vi "Control - Industrial Control.vi"() -> ()   [LabVIEW 2019, in "Control Workspace Object.lvlib"]
doc: "Sample numeric display item."
uses:
  Control Workspace Object.lvlib
  <vilib>/NI VeriStand/Display Template Support/DisplayTemplateSupport.llb/enum_Display Template Handler Minimal To Widget Msg.ctl
  <vilib>/NI VeriStand/Display Template Support/DisplayTemplateSupport.llb/enum_Display Template Handler Minimal To Workspace.ctl
  Addon/Addon Shared/SubVIs/Constants.vi
  Addon/Addon Shared/Control Addon Shared.lvlib
  Workspace Shared/Control Workspace Shared.lvlib
  Types/Workspace Object Cached Settings.ctl
  Types/Workspace Object State Variables.ctl
  <vilib>/NI VeriStand/Execution/Workspace/NI_VS Workspace ExecutionAPI.lvlib
  Workspace Shared/Types/UDP Streaming Command Cluster.ctl
  Workspace Shared/Types/UDP Streaming State.ctl
  <vilib>/NI VeriStand/Execution/Workspace/SystemStateRegEventRef.ctl
  <vilib>/NI VeriStand/Execution/Workspace/WorkspaceAPI.ctl
  <vilib>/NI VeriStand/Execution/Workspace/SystemStateEventRef.ctl
  Workspace Shared/Types/UI.Chart.Refs.ctl
  <vilib>/NI VeriStand/Execution/Workspace/Target State.ctl
  <vilib>/NI VeriStand/Execution/Workspace/Target State Info.ctl
  <vilib>/NI VeriStand/Execution/Workspace/NI VeriStand - Get Multiple Channel Values.vi
  <vilib>/NI VeriStand/Display Template Support/DisplayTemplateSupport.llb/sub_Display Template Handler Custom.vi
  <vilib>/NI VeriStand/Execution/Workspace/NI VeriStand - Set Single Channel Value.vi
  NationalInstruments.VeriStand.ClientAPI
  NationalInstruments.VeriStand.SystemStorage
  <vilib>/NI VeriStand/Display Template Support/DisplayTemplateSupport.llb/cluster_Screen Item Settings.ctl
  <vilib>/NI VeriStand/Display Template Support/DisplayTemplateSupport.llb/cluster_Graph Scale Settings.ctl
  <vilib>/NI VeriStand/Display Template Support/DisplayTemplateSupport.llb/cluster_Graph Plot Settings.ctl
panel:
  in  "Manual Value":bool
  in  "Revert":bool
  in  "Apply":bool
  in  "Manual Output":dbl
  in  "Manual Control":bool
  in  "Setpoint":dbl
  in  "NIVS.System Definition Root":refnum<k24>
  in  "NIVS.Gateway IP Address":string
  in  "Hold":bool
  in  "Autoscale Y":bool=TRUE
  in  "Autoscale X":bool=TRUE
  out "Chart":waveform(dbl)[](graph)
  out "Device":string
  in  "Item.Data":T1
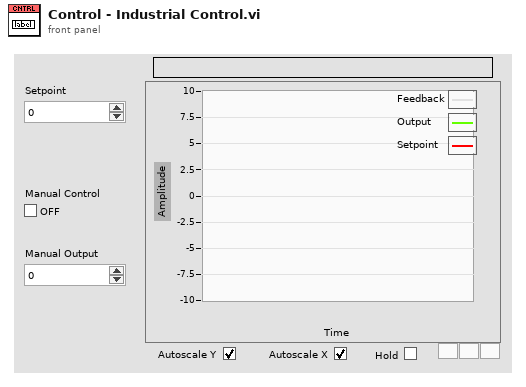
[diagram p1: front panel]
types:
  T1 = typedef "cluster_Screen Item Settings.ctl" = cluster{"Template VI":string, "Position X":i32, "Position Y":i32, "Custom":string, "Show Title Bar":bool, "ID":i32, "Always On Top":bool, "Allow Resize":bool, "Allow Minimize":bool, "Allow Close":bool, "Size to Screen":bool, "Screen.ID":i32, "State":enum16{"Normal", "New"}, "Title":string, "Window Bounds":cluster{"[0]":i16, "[1]":i16, "[2]":i16, "[3]":i16}, "Channel Ref":u64, "Unit":string, "Default Units?":bool, "Flash Limit?":bool, "Color 1":u32, "Color 2":u32, "Color 3":u32, "Color 4":u32, "Bck Color":u32, "Fore Color":u32, "Limit 1":dbl, "Limit 2":dbl, "Limit 3":dbl, "Limit 4":dbl, "Limit Mode 1":i32, "Limit Mode 2":i32, "Limit Mode 3":i32, "Limit Mode 4":i32, "Scale Precision":i32, "Scale Min":dbl, "Scale Max":dbl, "Format":i32, "Precision":i32, "Background Type":i32, "IDs":i32[], "Units":string[], "Labels":string[], "Scale Factor":dbl, "Scale Offset":dbl, "YScale Index":u32[], "XScale":T2, "YScales":T2[], "Plots":T3[], "Update Period":dbl, "History Length":dbl, "My.Ref":refnum<vi>, "Is Control?":bool, "Channel Paths":string[], "Custom Data":variant}
  T2 = typedef "cluster_Graph Scale Settings.ctl" = cluster{"Format":u8, "Precision":u8, "Fit":u8, "Label":string, "Use Default Label":bool, "Label Visible":bool, "Min":dbl, "Max":dbl}
  T3 = typedef "cluster_Graph Plot Settings.ctl" = cluster{"Bar Style":u8, "Fill To":i16, "Fill/PtColor":u32, "Line Style":u8, "Line Width":u8, "Color":u32, "Interp":u8, "Point Style":u8}
  T4 = typedef "Control Workspace Object.lvlib/Workspace Object State Variables.ctl" = cluster{"UI.Chart.Refs":T5, "Addon.GUID":string, "Addon.Name":string, "Addon.Type":enum16{"PID", "Industrial"}, "Data.UDPEngineQueue":refnum<queue>, "Data.Found?":bool, "Data.UDPChannels":string[], "Data.PreviousValues":dbl[], "Data.SlowChannels":string[], "Data.PendingChange?":bool, "CachedData.UserEvent":refnum<user-event>, "CachedData.Data":T6, "Addon.Connected?":bool, "NIVS.SysDefRoot":refnum<k24>, "NIVS.Workspace":T7, "NIVS.UserEventRefs":cluster{"Event Registration Refnum":refnum<event-registration>, "SystemChangeEventRef":T8}, "NIVS.SystemStateRefs":T9, "NIVS.LaunchRef":refnum<user-event>, "Setpoint Range":cluster{"Min":dbl, "Max":dbl}, "Output Range":cluster{"Min":dbl, "Max":dbl}, "UI.Device.Ref":refnum<vi>}
  T5 = typedef "Control Workspace Shared.lvlib/UI.Chart.Refs.ctl" = cluster{"Chart":refnum<vi>, "Manual Value":refnum<vi>, "Manual Output":refnum<vi>, "Revert":refnum<vi>, "Apply":refnum<vi>, "Setpoint":refnum<vi>, "Autoscale X":refnum<vi>, "Autoscale Y":refnum<vi>, "Hold":refnum<vi>, "Manual Control":refnum<vi>}
  T6 = typedef "Control Workspace Object.lvlib/Workspace Object Cached Settings.ctl" = cluster{"Path":string}
  T7 = typedef "NI_VS Workspace ExecutionAPI.lvlib/WorkspaceAPI.ctl" = refnum<k24>
  T8 = typedef "NI_VS Workspace ExecutionAPI.lvlib/SystemStateRegEventRef.ctl" = refnum<event-registration>
  T9 = typedef "NI_VS Workspace ExecutionAPI.lvlib/SystemStateEventRef.ctl" = cluster{"CustDatRef":refnum<user-event>, "EvtRef":refnum<k27>, "Target State User Event":refnum<user-event>}
  T10 = typedef "enum_Display Template Handler Minimal To Workspace.ctl" = cluster{"Operation":enum16{"SetCustomData", "DeleteItem"}, "Data":variant}
  T11 = typedef "enum_Display Template Handler Minimal To Widget Msg.ctl" = enum16{"Stop", "LaunchConfigDialog"}
  T12 = typedef "Control Workspace Shared.lvlib/UDP Streaming Command Cluster.ctl" = cluster{"Action":T13, "Channels":string[]}
  T13 = typedef "Control Workspace Shared.lvlib/UDP Streaming State.ctl" = enum8{"Idle", "Start Acq", "Run", "Stop Acq", "Exit"}
  T14 = cluster{"Event Registration Refnum":refnum<event-registration>, "SystemChangeEventRef":T8}
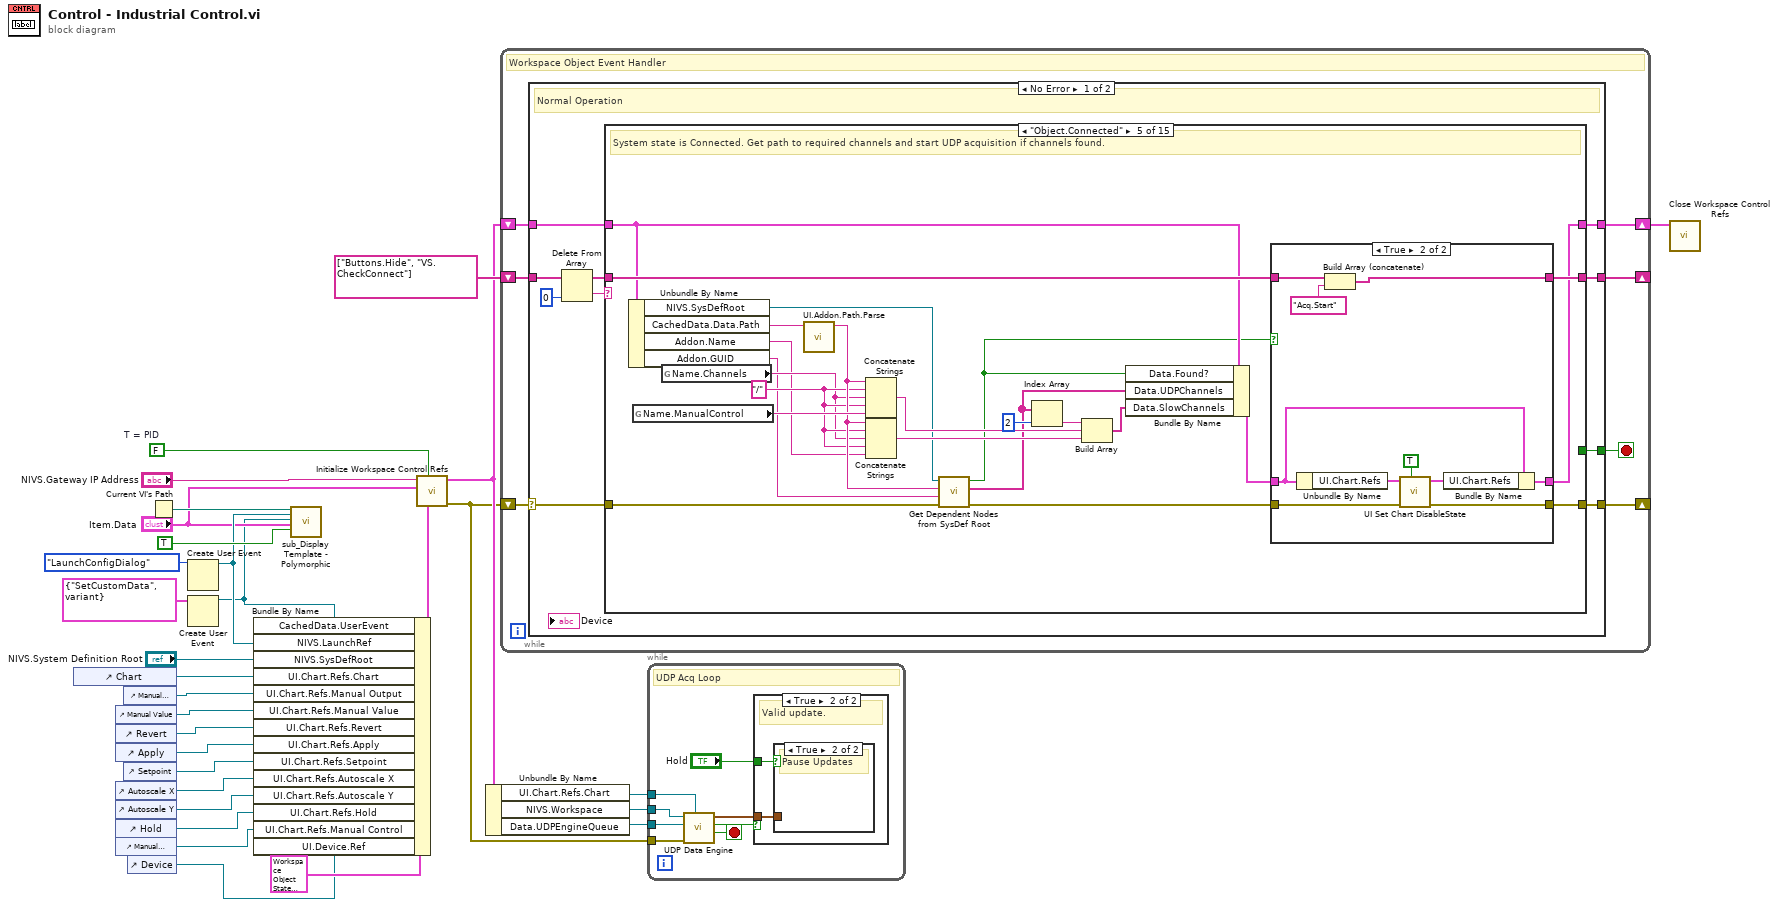
[diagram p0: block diagram]
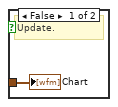
[diagram p3: hidden frame]
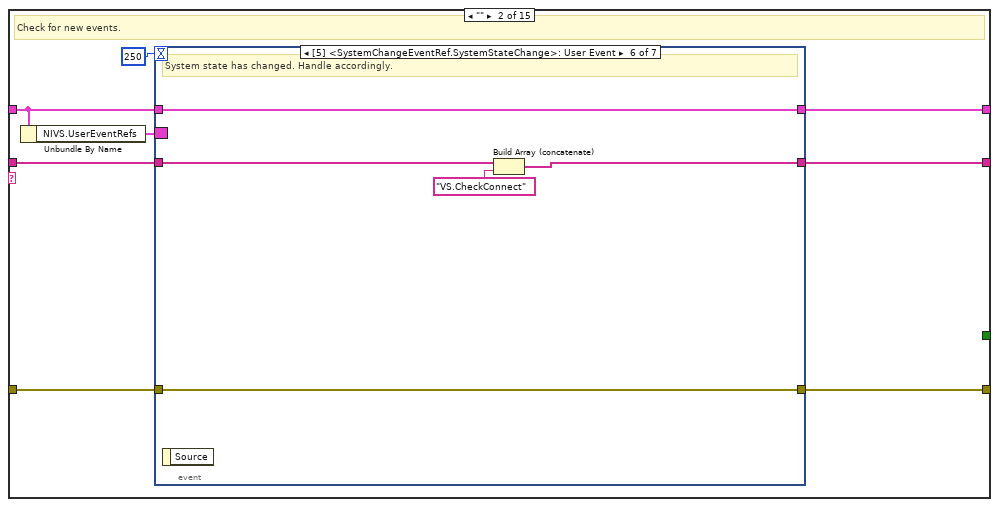
[diagram p5: hidden frame]
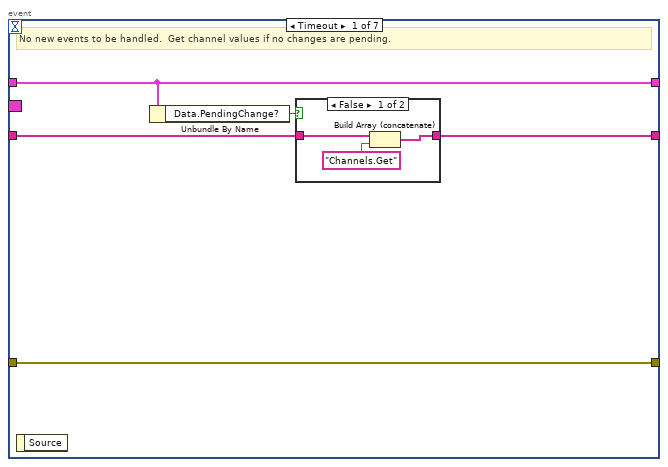
[diagram p6: hidden frame]
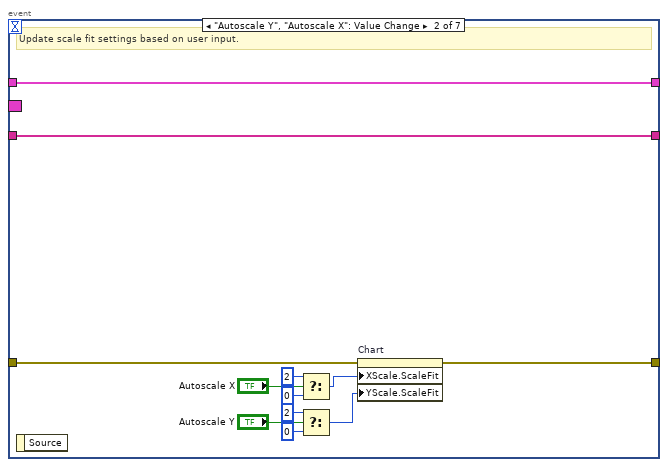
[diagram p8: hidden frame]
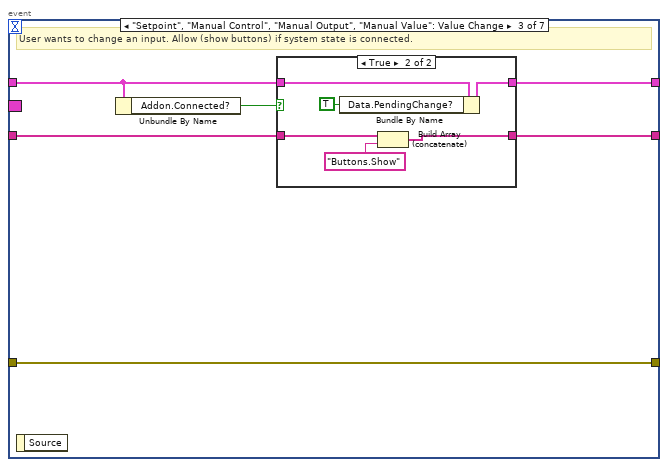
[diagram p9: hidden frame]
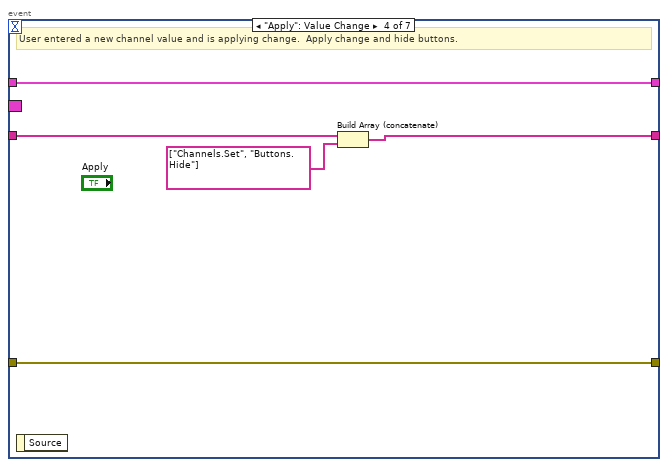
[diagram p11: hidden frame]
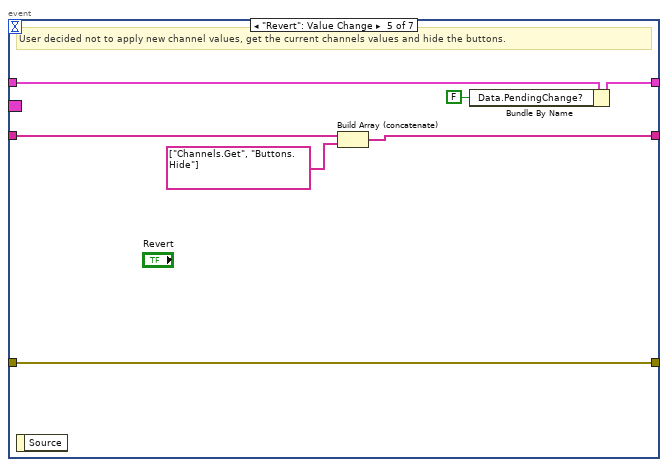
[diagram p12: hidden frame]
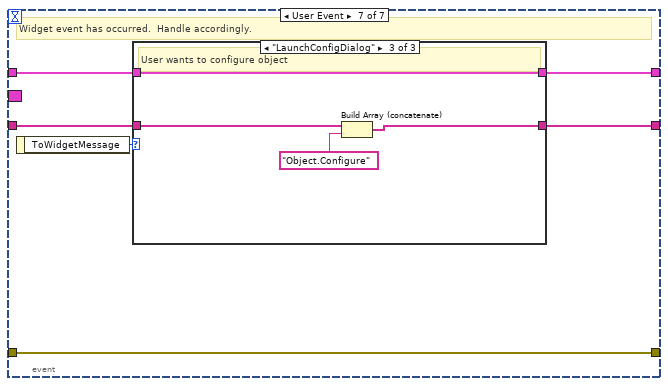
[diagram p13: hidden frame]
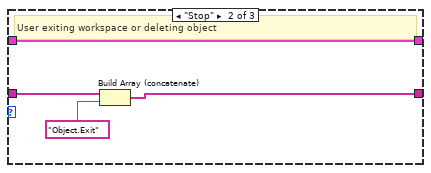
[diagram p15: hidden frame]
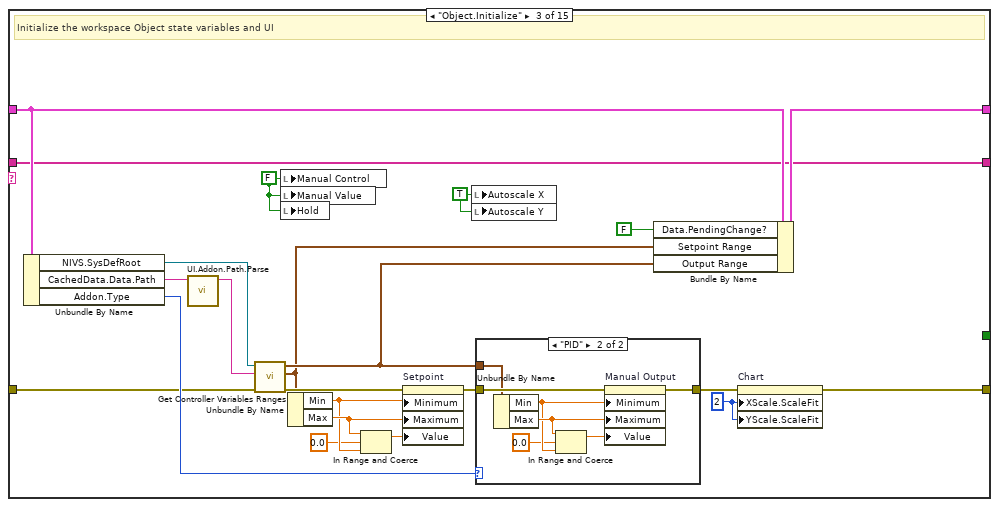
[diagram p16: hidden frame]
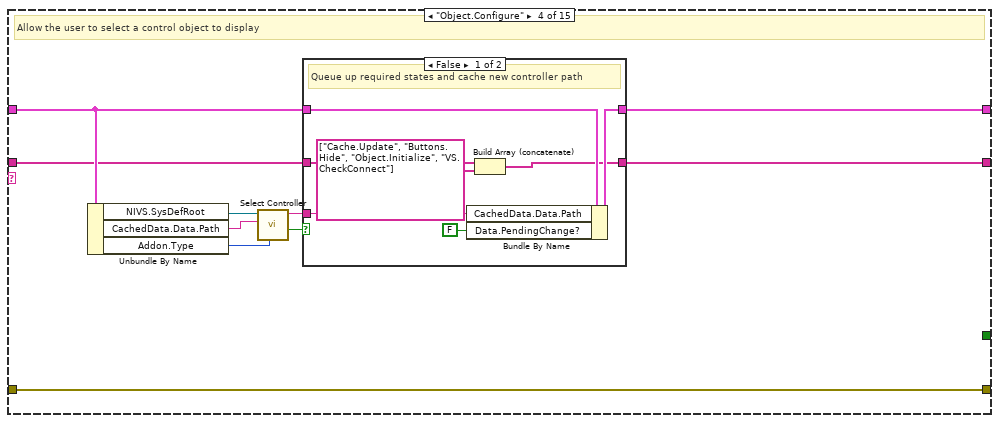
[diagram p18: hidden frame]
diagram:
  w13 = FALSE  # T = PID
  n1 = control-ref of="Chart"() -> (w19:refnum<vi>)
  n2 = control-ref of="Manual Value"() -> (w17:refnum<vi>)
  n3 = control-ref of="Revert"() -> (w16:refnum<vi>)
  n4 = control-ref of="Apply"() -> (w15:refnum<vi>)
  n5 = control-ref of="Autoscale X"() -> (w4:refnum<vi>)
  n6 = control-ref of="Autoscale Y"() -> (w5:refnum<vi>)
  n7 = control-ref of="Hold"() -> (w6:refnum<vi>)
  n8 = control-ref of="Manual Control"() -> (w3:refnum<vi>)
  n9 = control-ref of="Manual Output"() -> (w18:refnum<vi>)
  n10 = control-ref of="Setpoint"() -> (w7:refnum<vi>)
  n11 = control-ref of="Device"() -> (w1:refnum<vi>)
  n12 = Current VI's Path() -> (path=w28:path)
  n13 = Create User Event(user event datatype=enum_Display_Template_Handler_Minimal_To_Widget_Msg."LaunchConfigDialog" ("ToWidgetMessage")) -> (user event=w14:refnum<user-event>)  [unwired: 1 in, 1 out]
  n14 = Create User Event(user event datatype=T10 {"Operation"=enum."SetCustomData", "Data"=variant} ("Data")) -> (user event=w9:refnum<user-event>)  [unwired: 1 in, 1 out]
  n15 = Bundle By Name(cluster=T4 {"UI.Chart.Refs"={"Chart"=refnum, "Manual Value"=refnum, "Manual Output"=refnum, "Revert"=refnum, "Apply"=refnum, "Setpoint"=refnum, "Autoscale X"=refnum, "Autoscale Y"=refnum, "Hold"=refnum, "Manual Control"=refnum}, "Addon.GUID"="", "Addon.Name"="", "Addon.Type"=enum."PID", "Data.UDPEngineQueue"=refnum, "Data.Found?"=FALSE, "Data.UDPChannels"=[], "Data.PreviousValues"=[], "Data.SlowChannels"=[], "Data.PendingChange?"=FALSE, "CachedData.UserEvent"=refnum, "CachedData.Data"={"Path"=""}, "Addon.Connected?"=FALSE, "NIVS.SysDefRoot"=refnum, "NIVS.Workspace"=refnum, "NIVS.UserEventRefs"={"Event Registration Refnum"=refnum, "SystemChangeEventRef"=refnum}, "NIVS.SystemStateRefs"={"CustDatRef"=refnum, "EvtRef"=refnum, "Target State User Event"=refnum}, "NIVS.LaunchRef"=refnum, "Setpoint Range"={"Min"=0.0, "Max"=0.0}, "Output Range"={"Min"=0.0, "Max"=0.0}, "UI.Device.Ref"=refnum}, "CachedData.UserEvent"=w9, "NIVS.LaunchRef"=w14, "NIVS.SysDefRoot"="NIVS.System Definition Root", "UI.Chart.Refs.Chart"=w19, "UI.Chart.Refs.Manual Output"=w18, "UI.Chart.Refs.Manual Value"=w17, "UI.Chart.Refs.Revert"=w16, "UI.Chart.Refs.Apply"=w15, "UI.Chart.Refs.Setpoint"=w7, "UI.Chart.Refs.Autoscale X"=w4, "UI.Chart.Refs.Autoscale Y"=w5, "UI.Chart.Refs.Hold"=w6, "UI.Chart.Refs.Manual Control"=w3, "UI.Device.Ref"=w1) -> (w11:T4)
  n16 = call-poly <vilib>:"sub_Display Template - Polymorphic.vi"("Parent.Path"=w28, "ToWidgetEvent"=w14, "ToWorkspace"=w9, "Item.Data"="Item.Data", "Resizable"=TRUE) -> ()  [unwired: 1 in, 14 out]
  n17 = call "Initialize Workspace Control Refs.vi"("T = PID"=w13, "State Variables in"=w11, "Item.Data"="Item.Data", "NIVS.Gateway IP Address"="NIVS.Gateway IP Address") -> ("error out"=w8:errorcluster, "State Variables out"=w22:T4)  [unwired: 6 in]
  n18 = Unbundle By Name(w22) -> ("UI.Chart.Refs.Chart"=w24:refnum<vi>, "NIVS.Workspace"=w23:T7, "Data.UDPEngineQueue"=w21:refnum<queue>)
  n19 = while {
    shift-right: [w35] -> _
    shift-left: string[] ["Buttons.Hide", "VS.CheckConnect"] -> [w36]
    shift-right: [w33] -> w2
    shift-left: w22 -> [w32]
    shift-right: [w34] -> _
    shift-left: w8 -> [w31]
    stop <- w37 stop-if-true
    # "Workspace Object Event Handler"
    n20 = case shown="No Error" w31 {
      selector: w31 -> [w38 w386]
      tunnel: [w47 _] -> w37
      tunnel: w36 -> [w45 w394]
      tunnel: [w42 w394] -> w35
      tunnel: [w41 w391] -> w34
      tunnel: [w40 w393] -> w33
      tunnel: w32 -> [w39 w393]
      frame No Error {
        # "Normal Operation"
        n21 = Delete From Array(array=w45, index=0) -> (deleted portion=w44:string, array with subset deleted=w43:string[])  [unwired: 1 in]
        n22 = case shown="\"Object.Connected\"" w44 {
          tunnel: [_ _ _ _ _ _ _ TRUE _ _ _ _ _ _ _] -> w47
          tunnel: [w50 w57 w137 w160 w189 w219 w223 w249 w256 w264 w265 w276 w282 w297 w357] -> w42
          tunnel: w38 -> [w49 w55 w136 w166 w182 w216 w232 w244 w255 w259 w270 w272 w278 w294 w345]
          tunnel: w43 -> [w50 w56 w137 w159 w198 w219 w224 w249 w256 w264 w265 w276 w282 w297 w357]
          tunnel: w39 -> [w48 w51 w145 w164 w197 w214 w221 w241 w252 w263 w267 w275 w281 w287 w343]
          tunnel: [w49 w54 w144 w166 w177 w217 w233 w243 w255 w258 w269 w271 w277 w293 w344] -> w41
          tunnel: [w48 w53 w148 w163 w179 w212 w222 w241 w252 w263 w267 w275 w281 w292 w342] -> w40
          frame Default {
            # "Do nothing."
          }
          frame "" {
            # "Check for new events."
            n23 = Unbundle By Name(w51) -> ("NIVS.UserEventRefs"=w52:T14)
            n24 = event shown="[5] <SystemChangeEventRef.SystemStateChange>: User Event" {
              selector: w52 -> [_ _ _ _ _ _ _]
              dyn-events: _ -> [_ _ _ _ _ _ _]
              timeout: 250 -> [_ _ _ _ _ _ _]
              tunnel: [w61 w79 w82 w94 w102 w109 w115] -> w57
              tunnel: w56 -> [w62 w79 w83 w95 w103 w110 w114]
              tunnel: w55 -> [w63 w73 w85 w98 w105 w106 w113]
              tunnel: [w63 w72 w85 w98 w105 w106 w113] -> w54
              tunnel: [w60 w78 w84 w97 w100 w107 w111] -> w53
              tunnel: w51 -> [w60 w78 w81 w97 w101 w107 w112]
              event Timeout {
                # "No new events to be handled.  Get channel values if no changes are pending."
                n25 = event-data() -> ()  [unwired: 2 out]
                n26 = Unbundle By Name(w60) -> ("Data.PendingChange?"=w59:bool)
                n27 = case shown="False" w59 {
                  tunnel: w62 -> [w65 w67]
                  tunnel: [w64 w67] -> w61
                  frame False {
                    n28 = Build Array (concatenate)(w65, "Channels.Get") -> (w64:string[])
                  }
                  frame True {
                  }
                }
              }
              event "Autoscale Y", "Autoscale X": Value Change {
                # "Update scale fit settings based on user input."
                n29 = event-data() -> ()  [unwired: 2 out]
                n30 = Select(t=u8 2, s="Autoscale X", f=u8 0 ("X Scale.Scale Fit")) -> (s? t:f=w75:u8)
                n31 = Select(t=u8 2, s="Autoscale Y", f=u8 0 ("X Scale.Scale Fit")) -> (s? t:f=w68:u8)
                n32 = property on="Chart" class="WFChart (strict)"(error in=w73, "XScale.ScaleFit"=w75, "YScale.ScaleFit"=w68) -> (error out=w72:errorcluster)  [unwired: 1 in, 1 out]
              }
              event "Setpoint", "Manual Control", "Manual Output", "Manual Value": Value Change {
                # "User wants to change an input. Allow (show buttons) if system state is connected."
                n33 = event-data() -> ()  [unwired: 2 out]
                n34 = Unbundle By Name(w81) -> ("Addon.Connected?"=w80:bool)
                n35 = case shown="True" w80 {
                  tunnel: w81 -> [w86 w92]
                  tunnel: [w86 w91] -> w84
                  tunnel: w83 -> [w87 w90]
                  tunnel: [w87 w88] -> w82
                  frame False {
                  }
                  frame True {
                    n36 = Bundle By Name(cluster=w92, "Data.PendingChange?"=TRUE ("Pending Change?")) -> (w91:T4)
                    n37 = Build Array (concatenate)(w90, "Buttons.Show") -> (w88:string[])
                  }
                }
              }
              event "Apply": Value Change {
                # "User entered a new channel value and is applying change.  Apply change and hide buttons."
                n38 = event-data() -> ()  [unwired: 2 out]
                n39 = Build Array (concatenate)(w95, string[] ["Channels.Set", "Buttons.Hide"]) -> (w94:string[])
              }
              event "Revert": Value Change {
                # "User decided not to apply new channel values, get the current channels values and hide the buttons."
                n40 = event-data() -> ()  [unwired: 2 out]
                n41 = Build Array (concatenate)(w103, string[] ["Channels.Get", "Buttons.Hide"]) -> (w102:string[])
                n42 = Bundle By Name(cluster=w101, "Data.PendingChange?"=FALSE ("Pending Change?")) -> (w100:T4)
              }
              event User Event {
                # "System state has changed. Handle accordingly."
                n43 = event-data() -> ()  [unwired: 2 out]
                n44 = Build Array (concatenate)(w110, "VS.CheckConnect") -> (w109:string[])
              }
              event User Event {
                # "Widget event has occurred.  Handle accordingly."
                n45 = event-data() -> ("ToWidgetMessage"=w116:T11)  [unwired: 1 out]
                n46 = case shown="\"LaunchConfigDialog\"" w116 {
                  tunnel: [w118 w121 w125] -> w115
                  tunnel: w114 -> [w118 w122 w126]
                  tunnel: w112 -> [w117 w119 w123]
                  tunnel: [w117 w119 w123] -> w111
                  frame Default {
                    # "Do nothing."
                  }
                  frame "Stop" {
                    # "User exiting workspace or deleting object"
                    n47 = Build Array (concatenate)(w122, "Object.Exit") -> (w121:string[])
                  }
                  frame "LaunchConfigDialog" {
                    # "User wants to configure object"
                    n48 = Build Array (concatenate)(w126, "Object.Configure") -> (w125:string[])
                  }
                }
              }
            }
          }
          frame "Object.Initialize" {
            w131 = TRUE ("Manual Control")
            w132 = FALSE ("Manual Control")
            w147 = u8 2 ("X Scale.Scale Fit")
            # "Initialize the workspace Object state variables and UI"
            n49 = Unbundle By Name(w145) -> ("NIVS.SysDefRoot"=w133:refnum<k24>, "CachedData.Data.Path"=w135:string, "Addon.Type"=w140:enum16{"PID", "Industrial"})
            n50 = call "UI.Addon.Path.Parse.vi"("Cached Addon Path"=w135) -> ("Addon Path"=w134:string)  [unwired: 6 in, 4 out]
            n51 = call "Get Controller Variables Ranges.vi"("error in (no error)"=w136, "Path"=w134, "NIVS.SysDef Ref"=w133) -> ("error out"=w143:errorcluster, "Setpoint Range"=w138:cluster{"Min":dbl, "Max":dbl}, "Output Range"=w139:cluster{"Min":dbl, "Max":dbl})  [unwired: 6 in]
            n52 = local write "Manual Control"(w132) -> ()
            n53 = local write "Manual Value"(w132) -> ()
            n54 = local write "Hold"(w132) -> ()
            n55 = Unbundle By Name(w138) -> ("Min"=w129:dbl, "Max"=w130:dbl)
            n56 = In Range and Coerce(upper limit=w130, x=0.0, lower limit=w129) -> (coerced(x)=w128:dbl)  [unwired: 1 out]
            n57 = property on="Setpoint" class="DigNum (strict)"(error in=w143, "Minimum"=w129, "Maximum"=w130, "Value"=w128) -> (error out=w142:errorcluster)  [unwired: 1 in, 1 out]
            n58 = local write "Autoscale X"(w131) -> ()
            n59 = local write "Autoscale Y"(w131) -> ()
            n60 = case shown="\"PID\"" w140 {
              tunnel: w142 -> [w149 w156]
              tunnel: [w149 w155] -> w141
              tunnel: w139 -> [_ w154]
              frame Default {
              }
              frame "PID" {
                n61 = Unbundle By Name(w154) -> ("Min"=w152:dbl, "Max"=w153:dbl)
                n62 = In Range and Coerce(upper limit=w153, x=0.0, lower limit=w152) -> (coerced(x)=w150:dbl)  [unwired: 1 out]
                n63 = property on="Manual Output" class="DigNum (strict)"(error in=w156, "Minimum"=w152, "Maximum"=w153, "Value"=w150) -> (error out=w155:errorcluster)  [unwired: 1 in, 1 out]
              }
            }
            n64 = Bundle By Name(cluster=w145, "Data.PendingChange?"=FALSE ("Pending Change?"), "Setpoint Range"=w138, "Output Range"=w139) -> (w148:T4)
            n65 = property on="Chart" class="WFChart (strict)"(error in=w141, "XScale.ScaleFit"=w147, "YScale.ScaleFit"=w147) -> (error out=w144:errorcluster)  [unwired: 1 in, 1 out]
          }
          frame "Object.Configure" {
            # "Allow the user to select a control object to display"
            n66 = Unbundle By Name(w164) -> ("NIVS.SysDefRoot"=w158:refnum<k24>, "CachedData.Data.Path"=w165:string, "Addon.Type"=w157:enum16{"PID", "Industrial"})
            n67 = call "Select Controller.vi"("Type"=w157, "CD Path"=w165, "NIVS.System Definition Root"=w158) -> ("Cancelled?"=w162:bool, "Custom Device Path Out"=w161:string)  [unwired: 6 in, 1 out]
            n68 = case shown="False" w162 {
              tunnel: w164 -> [w173 w174]
              tunnel: [w172 w174] -> w163
              tunnel: w161 -> [w171 _]
              tunnel: [w169 w175] -> w160
              tunnel: w159 -> [w170 w175]
              frame False {
                # "Queue up required states and cache new controller path"
                n69 = Bundle By Name(cluster=w173, "CachedData.Data.Path"=w171, "Data.PendingChange?"=FALSE) -> (w172:T4)
                n70 = Build Array (concatenate)(w170, string[] ["Cache.Update", "Buttons.Hide", "Object.Initialize", "VS.CheckConnect"]) -> (w169:string[])
              }
              frame True {
                # "User canceled"
              }
            }
          }
          frame "Object.Connected" {
            w186 = "/" ("string")
            # "System state is Connected. Get path to required channels and start UDP acquisition if channels found."
            n71 = Unbundle By Name(w197) -> ("NIVS.SysDefRoot"=w183:refnum<k24>, "CachedData.Data.Path"=w196:string, "Addon.Name"=w184:string, "Addon.GUID"=w181:string)
            n72 = global read "Constants.vi" "Name.ManualControl"() -> (w195:string)
            n73 = global read "Constants.vi" "Name.Channels"() -> (w185:string)
            n74 = call "UI.Addon.Path.Parse.vi"("Cached Addon Path"=w196) -> ("Addon Path"=w194:string)  [unwired: 6 in, 4 out]
            n75 = Concatenate Strings(w194, w186, w185, w186, w195) -> (w193:string)
            n76 = Concatenate Strings(w194, w186, w185, w186, w184) -> (w192:string)
            n77 = call "Get Dependent Nodes from SysDef Root.vi"("error in (no error)"=w182, "GUID"=w181, "Path"=w194, "SysDef Ref"=w183) -> ("error out"=w178:errorcluster, "Channels"=w188:string[], "Found"=w176:bool)  [unwired: 5 in]
            n78 = Index Array(array=w188, index=2) -> (element=w190:string)
            n79 = Build Array(w190, w193, w192) -> (w187:string[])
            n80 = Bundle By Name(cluster=w197, "Data.Found?"=w176, "Data.UDPChannels"=w188, "Data.SlowChannels"=w187) -> (w180:T4)
            n81 = case shown="True" w176 {
              tunnel: w198 -> [w199 w211]
              tunnel: [w199 w210] -> w189
              tunnel: w180 -> [w200 w204]
              tunnel: [w200 w202] -> w179
              tunnel: w178 -> [w201 w209]
              tunnel: [w201 w208] -> w177
              frame False {
              }
              frame True {
                n82 = Unbundle By Name(w204) -> ("UI.Chart.Refs"=w205:T5)
                n83 = Build Array (concatenate)(w211, "Acq.Start") -> (w210:string[])
                n84 = call "UI Set Chart DisableState.vi"("Enable?"=TRUE, "error in (no error)"=w209, "UI.Chart.Refs"=w205) -> ("error out"=w208:errorcluster, "UI.Chart.Refs"=w203:T5)  [unwired: 7 in]
                n85 = Bundle By Name(cluster=w204, "UI.Chart.Refs"=w203) -> (w202:T4)
              }
            }
          }
          frame "Object.Disconnected" {
            n86 = Unbundle By Name(w214) -> ("UI.Chart.Refs"=w215:T5)
            n87 = call "UI Set Chart DisableState.vi"("Enable?"=FALSE, "error in (no error)"=w216, "UI.Chart.Refs"=w215) -> ("error out"=w217:errorcluster, "UI.Chart.Refs"=w213:T5)  [unwired: 7 in]
            n88 = Bundle By Name(cluster=w214, "UI.Chart.Refs"=w213) -> (w212:T4)
          }
          frame "VS.CheckConnect" {
            n89 = Unbundle By Name(w221) -> ("UI.Device.Ref"=w231:refnum<vi>, "NIVS.Workspace"=w230:T7, "NIVS.SysDefRoot"=w229:refnum<k24>, "CachedData.Data.Path"=w228:string)
            n90 = Current VI's Menubar() -> (w227:refnum<k9>)
            n91 = call "UI.Connection.State.Get.vi"("Menu Ref"=w227, "Name Ref"=w231, "error in (no error)"=w232, "Addon Path in"=w228, "NIVS.System Definition Root in"=w229, "NIVS.Workspace Ref in"=w230) -> ("error out"=w233:errorcluster, "Addon Connected?"=w220:bool, "NIVS.System Definition Root out"=w225:refnum<k24>, "NIVS.Workspace Ref out"=w226:T7)  [unwired: 1 in, 1 out]
            n92 = case shown="False" w220 {
              tunnel: w224 -> [w235 w238]
              tunnel: [w236 w239] -> w223
              frame True {
                n93 = Build Array (concatenate)(w235, "Object.Connected") -> (w236:string[])
              }
              frame False {
                n94 = Build Array (concatenate)(w238, "Object.Disconnected") -> (w239:string[])
              }
            }
            n95 = Bundle By Name(cluster=w221, "NIVS.Workspace"=w226, "NIVS.SysDefRoot"=w225, "Addon.Connected?"=w220) -> (w222:T4)
          }
          frame "Object.Exit" {
            # "Stop current loop.  Queue Stop Acq and Exit to UDP loop."
            n96 = Unbundle By Name(w241) -> ("Data.UDPEngineQueue"=w240:refnum<queue>)
            n97 = Enqueue Element(queue=w240, element=T12 {"Action"=enum."Stop Acq", "Channels"=[]}, error in (no error)=w244) -> (queue out=w247:refnum<queue>, error out=w245:errorcluster)  [unwired: 1 in, 1 out]
            n98 = Enqueue Element(queue=w247, element=T12 {"Action"=enum."Exit", "Channels"=[]}, error in (no error)=w245) -> (error out=w243:errorcluster)  [unwired: 1 in, 2 out]
          }
          frame "Cache.Update" {
            # "Cache any data needing to be permenantly stored with the workspace object."
            n99 = Unbundle By Name(w252) -> ("CachedData.UserEvent"=w250:refnum<user-event>, "CachedData.Data"=w251:T6)
            n100 = Bundle By Name(cluster=T10 {"Operation"=enum."SetCustomData", "Data"=variant} ("event data"), "Data"=w251) -> (w253:T10)
            n101 = Generate User Event(user event=w250, event data cluster=w253) -> ()  [unwired: 2 in, 2 out]
          }
          frame "Acq.Start" {
            # "Send a Start Acq command to the UDP Loop.  Include the channels to  monitor."
            n102 = Unbundle By Name(w263) -> ("Data.UDPEngineQueue"=w257:refnum<queue>, "Data.UDPChannels"=w261:string[])
            n103 = Bundle By Name(cluster=T12 {"Action"=enum."Start Acq", "Channels"=[]}, "Channels"=w261) -> (w260:T12)
            n104 = Enqueue Element(queue=w257, element=w260, error in (no error)=w259) -> (error out=w258:errorcluster)  [unwired: 1 in, 2 out]
          }
          frame "Acq.Disconnect" {
            # "Send Stop Acq to the UDP Acq Loop.  Reset the UI."
            n105 = Unbundle By Name(w267) -> ("Data.UDPEngineQueue"=w266:refnum<queue>)
            n106 = Enqueue Element(queue=w266, element=T12 {"Action"=enum."Stop Acq", "Channels"=[]}, error in (no error)=w270) -> (error out=w269:errorcluster)  [unwired: 1 in, 2 out]
          }
          frame "Buttons.Hide" {
            w273 = FALSE ("Hold")
            # "Hide the apply and revert buttons from the user."
            n107 = property on="Apply" class="Bool"(error in=w272, "Visible"=w273) -> (error out=w274:errorcluster)  [unwired: 1 in, 1 out]
            n108 = property on="Revert" class="Bool"(error in=w274, "Visible"=w273) -> (error out=w271:errorcluster)  [unwired: 1 in, 1 out]
          }
          frame "Buttons.Show" {
            w279 = TRUE ("Hold")
            # "Show the apply and revert buttons to the user."
            n109 = property on="Apply" class="Bool"(error in=w278, "Visible"=w279) -> (error out=w280:errorcluster)  [unwired: 1 in, 1 out]
            n110 = property on="Revert" class="Bool"(error in=w280, "Visible"=w279) -> (error out=w277:errorcluster)  [unwired: 1 in, 1 out]
          }
          frame "Channels.Get" {
            # "Get the current slow speed channel values from VeriStand if no pending change, data paths are valid and system state is connected."
            n111 = Unbundle By Name(w287) -> ("Setpoint Range.Max"=w286:dbl, "Setpoint Range.Min"=w285:dbl, "Data.PendingChange?"=w288:bool, "Output Range.Max"=w284:dbl, "Output Range.Min"=w283:dbl, "Addon.Type"=w291:enum16{"PID", "Industrial"}, "Data.Found?"=w295:bool, "Addon.Connected?"=w296:bool, "NIVS.Workspace"=w290:T7, "Data.SlowChannels"=w289:string[])
            n112 = case shown="False" w288 {
              tunnel: w296 -> [w319 _]
              tunnel: w295 -> [w313 _]
              tunnel: w294 -> [w310 w336]
              tunnel: [w309 w336] -> w293
              tunnel: [w308 w337] -> w292
              tunnel: w291 -> [w307 _]
              tunnel: w290 -> [w306 _]
              tunnel: w289 -> [w304 _]
              tunnel: w287 -> [w303 w337]
              tunnel: w286 -> [w301 _]
              tunnel: w285 -> [w300 _]
              tunnel: w284 -> [w299 _]
              tunnel: w283 -> [w298 _]
              frame False {
                # "No pending data change.  Allow for a get."
                n113 = Compound Arithmetic op=AND(w313, w319) -> (w314:bool)
                n114 = case shown="False" w314 {
                  tunnel: w310 -> [w329 w335]
                  tunnel: [w329 w334] -> w309
                  tunnel: w306 -> [w328 w333]
                  tunnel: [w328 w332] -> w305
                  tunnel: w304 -> [_ w331]
                  tunnel: [dbl[] [0.0, 0.0, 0.0] ("Values") w330] -> w318
                  frame False {
                    # "Do Nothing."
                  }
                  frame True {
                    # "Connected & paths valid"
                    n115 = call-poly <vilib>:"NI VeriStand - Get Channel Value.vi"("error in (no error)"=w335, "Channels"=w331, "WorkspaceManager in"=w333) -> ("error out"=w334:errorcluster, "Values"=w330:dbl[], "WorkspaceManager out"=w332:T7)  [unwired: 6 in]
                  }
                }
                n116 = Index Array(array=w318) -> (element #1=w317:dbl, element #2=w312:dbl, element #3=w311:dbl)  [unwired: 3 in]
                n117 = case shown="\"Industrial\"" w307 {
                  tunnel: w311 -> [w321 w326]
                  tunnel: w299 -> [_ w324]
                  tunnel: w298 -> [_ w323]
                  frame "Industrial" {
                    n118 = To Long Integer(number=w321) -> (32bit integer=w322:i32)
                    n119 = Not Equal To 0?(x=w322) -> (x != 0?=w320:bool)
                    n120 = local write "Manual Value"(w320) -> ()
                  }
                  frame "PID" {
                    n121 = In Range and Coerce(upper limit=w324, x=w326, lower limit=w323) -> (coerced(x)=w325:dbl)  [unwired: 1 out]
                    n122 = local write "Manual Output"(w325) -> ()
                  }
                }
                n123 = To Long Integer(number=w312) -> (32bit integer=w316:i32)
                n124 = In Range and Coerce(upper limit=w301, x=w317, lower limit=w300) -> (coerced(x)=w302:dbl)  [unwired: 1 out]
                n125 = Not Equal To 0?(x=w316) -> (x != 0?=w315:bool)
                n126 = local write "Setpoint"(w302) -> ()
                n127 = local write "Manual Control"(w315) -> ()
                n128 = Bundle By Name(cluster=w303, "NIVS.Workspace"=w305, "Data.PreviousValues"=w318) -> (w308:T4)
              }
              frame True {
                # "A change is pending.  Don't get channels as this would overwrite the pending change."
              }
            }
          }
          frame "Channels.Set" {
            # "Set Channels if data paths are valid and system state is connected and there is a change in the data value."
            n129 = Unbundle By Name(w343) -> ("Data.Found?"=w348:bool, "Addon.Connected?"=w351:bool, "Data.PreviousValues"=w350:dbl[], "Data.SlowChannels"=w352:string[], "NIVS.Workspace"=w340:T7, "Addon.Type"=w338:enum16{"PID", "Industrial"})
            n130 = case shown="\"PID\"" w338 {
              tunnel: [w359 "Manual Output"] -> w346
              frame "Industrial" {
                n131 = Boolean To (0,1)(Boolean="Manual Value") -> (0, 1=w359:i16)
              }
              frame "PID" {
              }
            }
            n132 = Boolean To (0,1)(Boolean="Manual Control") -> (0, 1=w347:i16)
            n133 = Build Array("Setpoint", w347, w346) -> (w353:dbl[])
            n134 = Not Equal?(x=w350, y=w353) -> (x != y?=w356:bool[])
            n135 = Compound Arithmetic op=AND(w348, w351) -> (w349:bool)
            n136 = case shown="True" w349 {
              tunnel: w356 -> [_ w369]
              tunnel: w353 -> [_ w368]
              tunnel: w345 -> [w362 w367]
              tunnel: [w362 w366] -> w344
              tunnel: w340 -> [w361 w365]
              tunnel: [w361 w364] -> w339
              tunnel: w352 -> [_ w363]
              frame False {
                # "Do nothing"
              }
              frame True {
                # "Connected & paths valid"
                n137 = for {
                  shift-right: [w375] -> w366
                  shift-left: w367 -> [w376]
                  shift-right: [w374] -> w364
                  shift-left: w365 -> [w373]
                  tunnel: w369 -> [w372] mode=indexing
                  tunnel: w368 -> [w371] mode=indexing
                  tunnel: w363 -> [w370] mode=indexing
                  n138 = case shown="True" w372 {
                    tunnel: w376 -> [w378 w384]
                    tunnel: [w378 w383] -> w375
                    tunnel: [w377 w382] -> w374
                    tunnel: w373 -> [w377 w381]
                    tunnel: w371 -> [_ w380]
                    tunnel: w370 -> [_ w379]
                    frame False {
                      # "Do nothing"
                    }
                    frame True {
                      # "Update channel"
                      n139 = call-poly <vilib>:"NI VeriStand - Set Channel Value.vi"("error in (no error)"=w384, "Value"=w380, "Channel"=w379, "WorkspaceManager in"=w381) -> ("error out"=w383:errorcluster, "WorkspaceManager out"=w382:T7)  [unwired: 6 in]
                    }
                  }
                }
              }
            }
            n140 = Bundle By Name(cluster=w343, "Data.PendingChange?"=FALSE ("Pending Change?"), "NIVS.Workspace"=w339) -> (w342:T4)
          }
        }
      }
      frame Error {
        # "Handle Errors."
        n141 = Unbundle By Name(w386) -> ("code"=w390:i32)
        n142 = Equal?(x=-307654, y=w390) -> (x = y?=w388:bool)
        n143 = Select(t=errorcluster {"status"=FALSE, "code"=0, "source"=""}, s=w388, f=w386) -> (s? t:f=w385:errorcluster)
        n144 = call <vilib>:"Simple Error Handler.vi"("error in (no error)"=w385) -> ("error out"=w392:errorcluster)  [unwired: 4 in, 4 out]
        n145 = call <vilib>:"Clear Errors.vi"("error in (no error)"=w392) -> ("error out"=w391:errorcluster)  [unwired: 5 in, 1 out]
      }
    }
  }
  n146 = while {
    tunnel: w23 -> [w397]
    tunnel: w21 -> [w402]
    tunnel: w24 -> [w398]
    tunnel: w8 -> [w396]
    stop <- w401 stop-if-true
    # "UDP Acq Loop"
    n147 = call "UDP Data Engine.vi"("WaveformChart Ref"=w398, "error in (no error)"=w396, "UDP Engine Queue"=w402, "WorkspaceManager"=w397) -> ("Exit"=w401:bool, "Update?"=w395:bool, "Waveform"=w399:waveform(dbl)[])  [unwired: 4 in, 1 out]
    n148 = case shown="True" w395 {
      tunnel: "Hold" -> [_ w404]
      tunnel: w399 -> [_ w403]
      frame False {
        # "Do Nothing."
      }
      frame True {
        # "Valid update."
        n149 = case shown="True" w404 {
          tunnel: w403 -> [w405 _]
          frame False {
            # "Update."
            "Chart" <- w405
          }
          frame True {
            # "Pause Updates"
          }
        }
      }
    }
  }
  n150 = call "Close Workspace Control Refs.vi"("State Variables in"=w2) -> ()  [unwired: 11 in]
